vi "DAC Init Results.vi"(8 "error in":errorcluster, 9 "Log Details?":bool, 10 "tdms file":refnum<k34>, 11 "DAC HMP4040 in":refnum<class "DAC HMP4040.lvclass">) -> (0 "error out":errorcluster, 2 "tdms file out":refnum<k34>)   [LabVIEW 2019, in "DAC.lvlib" / "DAC HMP4040.lvclass"]
uses:
  DAC HMP4040.lvclass
  C:/Users/krio/Documents/LV_Projects/test-stand/App/DAC/DAC.lvclass
  DAC.lvclass/DAC.ctl
  DAC HMP4040.lvclass/DAC HMP4040.ctl
  DAC.lvclass
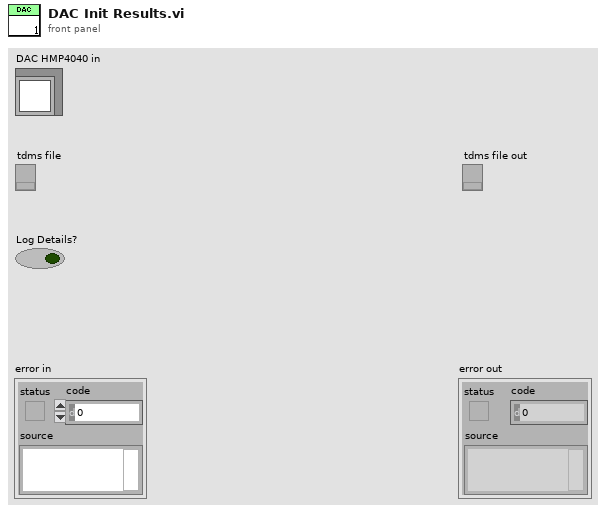
[diagram p1: front panel]
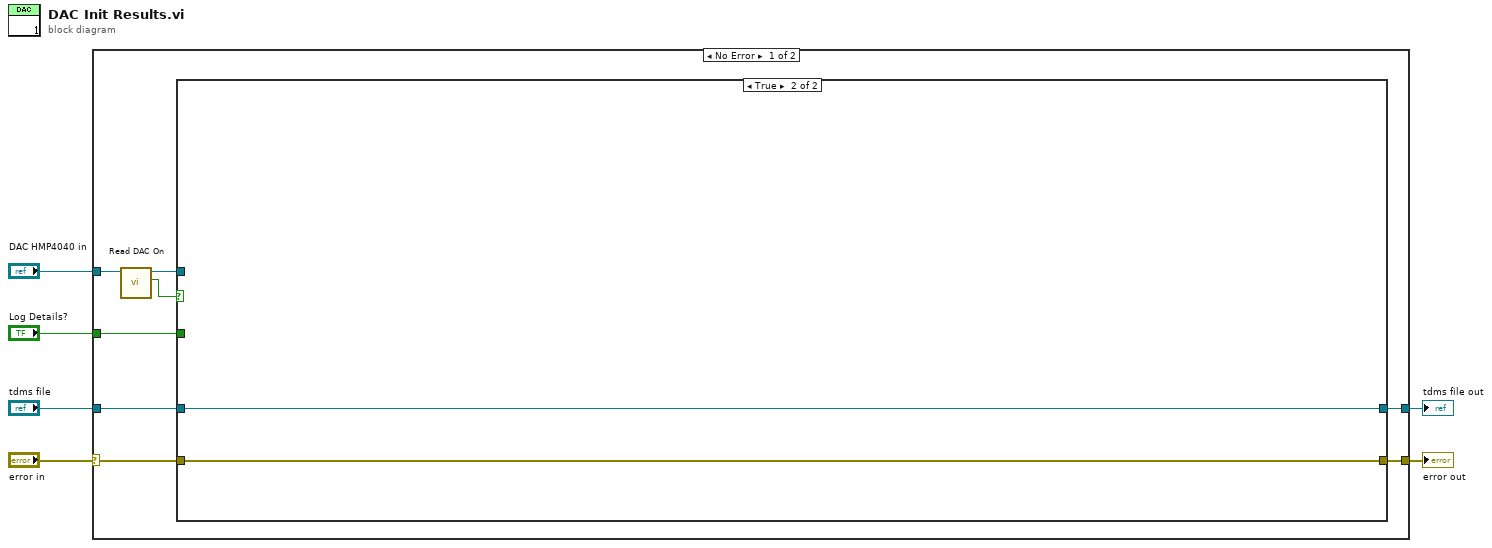
[diagram p0: block diagram]
diagram:
  n1 = case shown="No Error" "error in" {
    selector: "error in" -> [w8 w20]
    tunnel: [w12 w20] -> w3
    tunnel: "DAC HMP4040 in" -> [w11 _]
    tunnel: "tdms file" -> [w14 w19]
    tunnel: [w13 w19] -> w2
    tunnel: "Log Details?" -> [w7 _]
    frame No Error {
      n2 = call "Read DAC On.vi"("DAC in"=w11) -> ("DAC On"=w9:bool, "DAC out"=w10:refnum<class "DAC HMP4040.lvclass">)  [unwired: 8 in, 1 out]
      n3 = case shown="True" w9 {
        tunnel: w14 -> [w16 w18]
        tunnel: [w16 w18] -> w13
        tunnel: [w15 w17] -> w12
        tunnel: w10 -> [_ _]
        tunnel: w8 -> [w15 w17]
        tunnel: w7 -> [_ _]
        frame False {
        }
        frame True {
        }
      }
    }
    frame Error {
    }
  }
  "error out" <- w3
  "tdms file out" <- w2
